vi "Example.vi"() -> ()   [LabVIEW 2018]
uses:
  XButton/button3.xctl
panel:
  in  "风格四":bool(xcontrol)
  in  "风格三":bool(xcontrol)
  in  "风格二":bool(xcontrol)
  in  "风格一":bool(xcontrol)
  in  "按钮颜色盒":u32(colorbox)
  in  "背景颜色盒":u32(colorbox)
  out "数字(0-1)":u8
  # "LabVIEW实现按钮悬停动画效果"
  # "Click:"
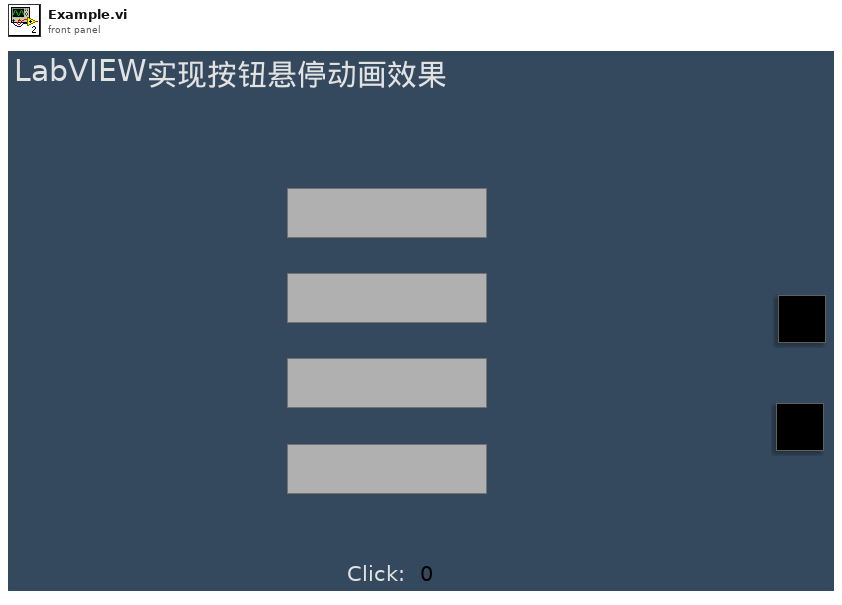
[diagram p1: front panel]
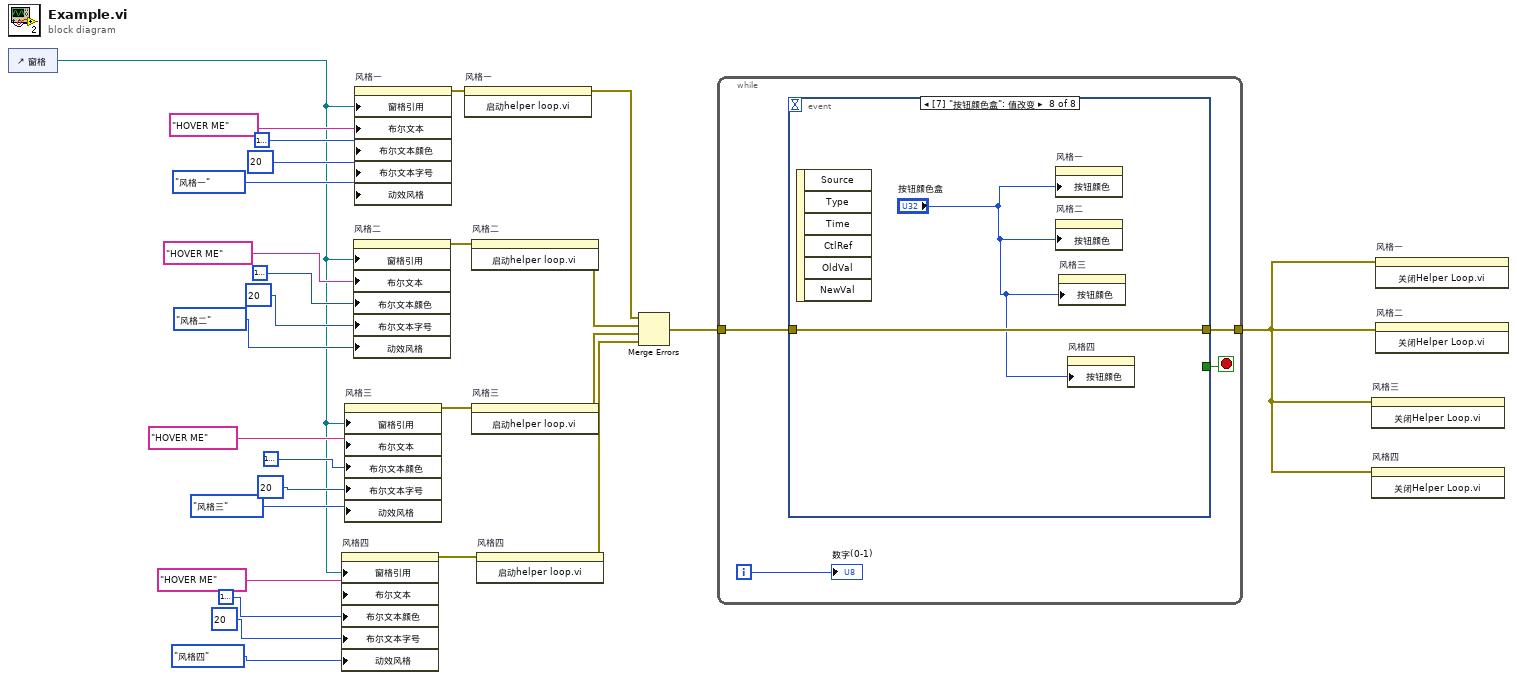
[diagram p0: block diagram]
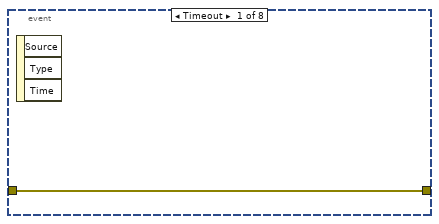
[diagram p2: hidden frame]
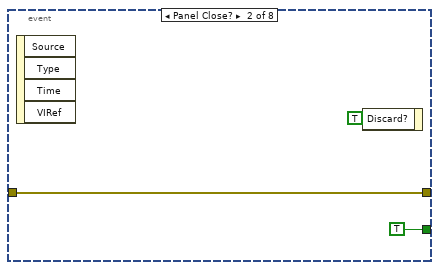
[diagram p3: hidden frame]
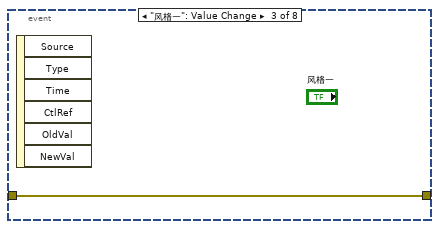
[diagram p4: hidden frame]
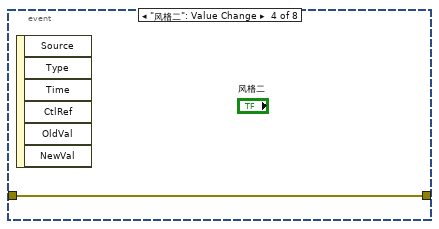
[diagram p5: hidden frame]
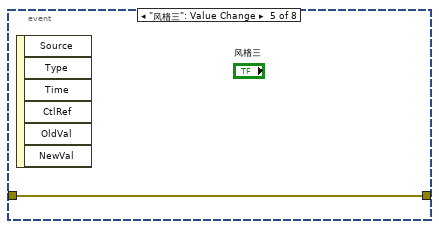
[diagram p6: hidden frame]
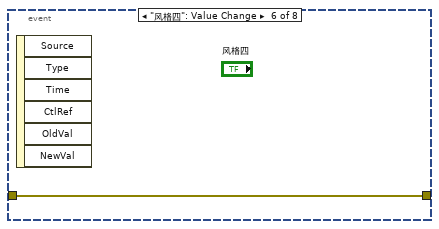
[diagram p7: hidden frame]
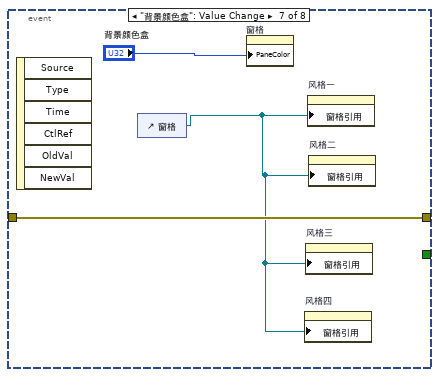
[diagram p8: hidden frame]
diagram:
  n1 = control-ref of="窗格"() -> (w8:refnum<vi>)
  n2 = property on="风格四" class="button3 (严格)"("窗格引用"=w8, "布尔文本"="HOVER ME", "布尔文本颜色"=u32 16777225, "布尔文本字号"=u32 20, "动效风格"=enum16{"风格一", "风格二", "风格三", "风格四"}."风格四") -> (error out=w3:errorcluster)  [unwired: 2 in, 1 out]
  n3 = property on="风格三" class="button3 (严格)"("窗格引用"=w8, "布尔文本"="HOVER ME", "布尔文本颜色"=u32 16777225, "布尔文本字号"=u32 20, "动效风格"=enum16{"风格一", "风格二", "风格三", "风格四"}."风格三") -> (error out=w10:errorcluster)  [unwired: 2 in, 1 out]
  n4 = property on="风格二" class="button3 (严格)"("窗格引用"=w8, "布尔文本"="HOVER ME", "布尔文本颜色"=u32 16777225, "布尔文本字号"=u32 20, "动效风格"=enum16{"风格一", "风格二", "风格三", "风格四"}."风格二") -> (error out=w16:errorcluster)  [unwired: 2 in, 1 out]
  n5 = property on="风格一" class="button3 (严格)"("窗格引用"=w8, "布尔文本"="HOVER ME", "布尔文本颜色"=u32 16777225, "布尔文本字号"=u32 20, "动效风格"=enum16{"风格一", "风格二", "风格三", "风格四"}."风格一") -> (error out=w22:errorcluster)  [unwired: 2 in, 1 out]
  n6 = invoke on="风格一" class="button3 (严格)" method="启动helper loop.vi"(error in=w22) -> (error out=w21:errorcluster)  [unwired: 2 in, 2 out]
  n7 = invoke on="风格二" class="button3 (严格)" method="启动helper loop.vi"(error in=w16) -> (error out=w15:errorcluster)  [unwired: 2 in, 2 out]
  n8 = invoke on="风格三" class="button3 (严格)" method="启动helper loop.vi"(error in=w10) -> (error out=w9:errorcluster)  [unwired: 2 in, 2 out]
  n9 = invoke on="风格四" class="button3 (严格)" method="启动helper loop.vi"(error in=w3) -> (error out=w2:errorcluster)  [unwired: 2 in, 2 out]
  n10 = Merge Errors(w21, w15, w9, w2) -> (w27:errorcluster)
  n11 = while {
    tunnel: w27 -> [w30]
    tunnel: [w29] -> w1
    i -> [w28]
    stop <- w31 stop-if-true
    n12 = event shown="[7] \"按钮颜色盒\": 值改变" {
      selector: _ -> [_ _ _ _ _ _ _ _]
      dyn-events: _ -> [_ _ _ _ _ _ _ _]
      timeout: _ -> [_ _ _ _ _ _ _ _]
      tunnel: [_ TRUE _ _ _ _ _ _] -> w31
      tunnel: w30 -> [w32 w33 w36 w37 w38 w39 w41 w44]
      tunnel: [w32 w33 w36 w37 w38 w39 w41 w44] -> w29
      event Timeout {
        n13 = event-data() -> ()  [unwired: 1 in, 3 out]
      }
      event Panel Close? {
        n14 = event-data() -> ()  [unwired: 1 in, 4 out]
        n15 = event-data("Discard?"=TRUE ("放弃？")) -> ()  [unwired: 1 in, 1 out]
      }
      event "风格一": Value Change {
        n16 = event-data() -> ()  [unwired: 1 in, 6 out]
      }
      event "风格二": Value Change {
        n17 = event-data() -> ()  [unwired: 1 in, 6 out]
      }
      event "风格三": Value Change {
        n18 = event-data() -> ()  [unwired: 1 in, 6 out]
      }
      event "风格四": Value Change {
        n19 = event-data() -> ()  [unwired: 1 in, 6 out]
      }
      event "背景颜色盒": Value Change {
        n20 = event-data() -> ()  [unwired: 1 in, 6 out]
        n21 = control-ref of="窗格"() -> (w40:refnum<vi>)
        n22 = property on="窗格" class="Pane"("PaneColor"="背景颜色盒") -> ()  [unwired: 2 in, 2 out]
        n23 = property on="风格四" class="button3 (严格)"("窗格引用"=w40) -> ()  [unwired: 2 in, 2 out]
        n24 = property on="风格三" class="button3 (严格)"("窗格引用"=w40) -> ()  [unwired: 2 in, 2 out]
        n25 = property on="风格一" class="button3 (严格)"("窗格引用"=w40) -> ()  [unwired: 2 in, 2 out]
        n26 = property on="风格二" class="button3 (严格)"("窗格引用"=w40) -> ()  [unwired: 2 in, 2 out]
      }
      event "按钮颜色盒": Value Change {
        n27 = event-data() -> ()  [unwired: 1 in, 6 out]
        n28 = property on="风格一" class="button3 (严格)"("按钮颜色"="按钮颜色盒") -> ()  [unwired: 2 in, 2 out]
        n29 = property on="风格二" class="button3 (严格)"("按钮颜色"="按钮颜色盒") -> ()  [unwired: 2 in, 2 out]
        n30 = property on="风格三" class="button3 (严格)"("按钮颜色"="按钮颜色盒") -> ()  [unwired: 2 in, 2 out]
        n31 = property on="风格四" class="button3 (严格)"("按钮颜色"="按钮颜色盒") -> ()  [unwired: 2 in, 2 out]
      }
    }
    "数字(0-1)" <- w28
  }
  n32 = invoke on="风格三" class="button3 (严格)" method="关闭Helper Loop.vi"(error in=w1) -> ()  [unwired: 2 in, 3 out]
  n33 = invoke on="风格四" class="button3 (严格)" method="关闭Helper Loop.vi"(error in=w1) -> ()  [unwired: 2 in, 3 out]
  n34 = invoke on="风格一" class="button3 (严格)" method="关闭Helper Loop.vi"(error in=w1) -> ()  [unwired: 2 in, 3 out]
  n35 = invoke on="风格二" class="button3 (严格)" method="关闭Helper Loop.vi"(error in=w1) -> ()  [unwired: 2 in, 3 out]
